vi "Async Loop.vi"(1 "RT Data":T1={"Device ref"=0, "Scan Period (uSec)"=10000, "Device Channels"={"Status"={"BD Refs"=[], "Length"=0, "FIFO Index"=0, "Data"=[]}, "Command"={"BD Refs"=[], "Data"=[], "Length"=0, "FIFO Index"=0}}, "Local Chassis"=[], "EtherCAT Masters"=[], "Async"={"Status"=refnum, "Command"=refnum, "Input FIFO"=refnum, "Input FIFO buffer"=[], "Output FIFO"=refnum, "Output FIFO buffer"=[], "Async VI Ref"=refnum}, "ECAT Reconfig"={"Reconfig Module Found"=FALSE, "VI Ref"=refnum, "Status"=refnum}, "Device Error"={"status"=FALSE, "code"=0, "source"=""}, "DeviceName"="", "PCLSync?"=FALSE} {"Device Channels"."Status"."BD Refs"."Data Reference" format="%.0x"; "Device Channels"."Command"."BD Refs"."Data Reference" format="%.0x"; "Local Chassis"."FPGA"."VS ref" format="%.0x"; "Local Chassis"."RSI Modules"."VS ref" format="%.0x"; "Local Chassis"."VS ref" format="%.0x"; "Device ref" format="%.0x"; "EtherCAT Masters"."REM IO ECAT Slaves"."VS ref" format="%.0x"; "EtherCAT Masters"."Generic EtherCAT Slaves"."VS ref" format="%.0x"; "EtherCAT Masters"."VS ref" format="%.0x"; "EtherCAT Masters"."EtherCAT Slaves"."FPGA"."VS ref" format="%.0x"; "EtherCAT Masters"."EtherCAT Slaves"."RSI Modules"."VS ref" format="%.0x"; "EtherCAT Masters"."EtherCAT Slaves"."VS ref" format="%.0x"}) -> ()   [LabVIEW 2020, in "SEECD Engine.lvlib"]
uses:
  SEECD Engine.lvlib
  <vilib>/Platform/TimedLoop/XDataNode/XDataNode.xnode
  <vilib>/Platform/TimedLoop/XDataNode/nitl_modes.ctl
  <vilib>/Platform/TimedLoop/XDataNode/XDNodeRunTimeDep.lvlib
  <vilib>/Platform/TimedLoop/XDataNode/wakeup.ctl
  <vilib>/Platform/TimedLoop/XDataNode/timing_clust.ctl
  <vilib>/NI VeriStand/Custom Device API/Custom Device API.lvlib
  <vilib>/NI VeriStand/Custom Device API/Custom Device Timed Loop Priority.ctl
  Type Defs/Async State.ctl
  Shared/Globals/String Constants.vi
  Shared/SEECD Shared.lvlib
  Type Defs/RW Case.ctl
  Type Defs/Async Command.ctl
  <vilib>/Platform/TimedLoop/XDataNode/loadnilvce.vi
  <vilib>/NI VeriStand/Custom Device Tools/Custom Device Utility Library/Custom Device Utility Library.lvlib
  <vilib>/NI VeriStand/Custom Device API/Custom Device Item Ref.ctl
  Includes/Modules.lvlibp/RSI Module/RSI Module.lvclass
  <vilib>/NI VeriStand/Custom Device API/Data Reference.ctl
  <vilib>/NI VeriStand/Custom Device API/Block Data Reference.ctl
  Type Defs/Input Data.ctl
  Type Defs/Output Data.ctl
  Includes/Modules.lvlibp/RSI Module/Channel Type.ctl
  Type Defs/RSI Module Data.ctl
  Type Defs/FPGA Data.ctl
  Type Defs/Local Chassis Data.ctl
  Type Defs/EtherCAT Slave Data.ctl
  Type Defs/EtherCAT Master Data.ctl
  Type Defs/RT Data.ctl
  Type Defs/Async Status.ctl
  Shared/Type Defs/UDV Data Type.ctl
  Shared/Type Defs/FXP Config.ctl
  Type Defs/UDV Data.ctl
  Includes/Modules.lvlibp/RSI Module/Module Models.ctl
  Type Defs/Module Config Data.ctl
  Type Defs/Async Data.ctl
  Type Defs/ECAT Reconfig State.ctl
  Type Defs/ECAT Reconfig Status.ctl
  Type Defs/ECAT Reconfig Data.ctl
  Type Defs/Device Channels.ctl
  Type Defs/Mixed IO.ctl
  Type Defs/Open Module IOVs.ctl
  Type Defs/Mod Size Indexes.ctl
  Type Defs/Generic ECAT Slave IOV Cluster.ctl
  Type Defs/Generic ECAT Slave Data Cluster.ctl
  Type Defs/Generic ECAT Slave RT-Data-Array.ctl
  Type Defs/REM IO ECAT Slave IOV Cluster.ctl
  Type Defs/REM IO ECAT Slave Data Cluster.ctl
  Type Defs/REM IO ECAT Slave RT-Data-Array.ctl
types:
  T1 = typedef "SEECD Engine.lvlib/RT Data.ctl" = cluster{"Device ref":T2, "Scan Period (uSec)":u32, "Device Channels":T3, "Local Chassis":T8[], "EtherCAT Masters":T20[], "Async":T28, "ECAT Reconfig":T29, "Device Error":errorcluster, "DeviceName":string, "PCLSync?":bool}
  T2 = typedef "Custom Device API.lvlib/Custom Device Item Ref.ctl" = u64
  T3 = typedef "SEECD Engine.lvlib/Device Channels.ctl" = cluster{"Status":T4, "Command":T7}
  T4 = typedef "SEECD Engine.lvlib/Output Data.ctl" = cluster{"BD Refs":T5[], "Length":i32, "FIFO Index":i32, "Data":dbl[]}
  T5 = typedef "Custom Device API.lvlib/Block Data Reference.ctl" = cluster{"Data Reference":T6, "Offset":u64, "Length":u64}
  T6 = typedef "Custom Device API.lvlib/Data Reference.ctl" = i32
  T7 = typedef "SEECD Engine.lvlib/Input Data.ctl" = cluster{"BD Refs":T5[], "Data":dbl[], "Length":i32, "FIFO Index":i32}
  T8 = typedef "SEECD Engine.lvlib/Local Chassis Data.ctl" = cluster{"VS ref":T2, "RSI Modules":T9[], "FPGA":T15[], "Input Mod Size Idxs":T19, "Output Modules":i32[], "MixedIO Mod Size Idxs":T19}
  T9 = typedef "SEECD Engine.lvlib/RSI Module Data.ctl" = cluster{"VS ref":T2, "IOV ref":refnum<k21>, "Open Mod refs":T10, "Module DVR":refnum<data-value>, "Slot":u32, "Model":T11, "Channel Type":T12, "EtherCAT?":bool, "CDInput Data":T7, "CDOutput Data":T4, "Module Config Data":T13, "Mixed IO":T14}
  T10 = typedef "SEECD Engine.lvlib/Open Module IOVs.ctl" = cluster{"Analog Read":refnum<k21>, "Digital Read":refnum<k21>, "Analog Write":refnum<k21>, "Digital Write":refnum<k21>}
  T11 = typedef "Modules.lvlibp/RSI Module.lvclass/Module Models.ctl" = enum16{"Empty", "NI 9201", "NI 9203", "NI 9205", "NI 9206", "NI 9207", "NI 9208", "NI 9209", "NI 9210", "NI 9211", "NI 9212", "NI 9213", "NI 9214", "NI 9215", "NI 9216", "NI 9217", "NI 9219", "NI 9220", "NI 9221", "NI 9222", "NI 9223", "NI 9224", "NI 9225", "NI 9226", "NI 9227", "NI 9228", "NI 9229", "NI 9233", "NI 9234", "NI 9235", "NI 9236", "NI 9237", "NI 9239", "NI 9242", "NI 9244", "NI 9253", "NI 9263", "NI 9264", "NI 9265", "NI 9266", "NI 9269", "NI 9344", "NI 9350", "NI 9375", "NI 9401", "NI 9402", "NI 9403", "NI 9411", "NI 9421", "NI 9422", "NI 9423", "NI 9425", "NI 9426", "NI 9435", "NI 9436", "NI 9437", "NI 9472", "NI 9474", "NI 9475", "NI 9476", "NI 9477", "NI 9478", "NI 9481", "NI 9482", "NI 9485"}
  T12 = typedef "Modules.lvlibp/RSI Module.lvclass/Channel Type.ctl" = enum16{"Analog", "Digital"}
  T13 = typedef "SEECD Engine.lvlib/Module Config Data.ctl" = cluster{"Configurable?":bool, "Config Block Data Refs":T5[], "Config Data DVR":refnum<data-value>, "Previous Values":dbl[], "Local Reconfig VI Ref":refnum<vi>}
  T14 = typedef "SEECD Engine.lvlib/Mixed IO.ctl" = cluster{"Input Channel Indices":i32[], "Input Buffer":dbl[]}
  T15 = typedef "SEECD Engine.lvlib/FPGA Data.ctl" = cluster{"VS ref":T2, "IOV ref":refnum<k21>, "FPGA Target":enum16{"Local", "EtherCAT"}, "Product Code":u32, "Bitfile Signature":string, "Bitfile Path (RT)":path, "FPGA Session":u32, "Input Data":T7, "Output Data":T4, "UDVs":cluster{"From FPGA":T16[], "To FPGA":T16[]}}
  T16 = typedef "SEECD Engine.lvlib/UDV Data.ctl" = cluster{"VS ref":T2, "IOV Ref":refnum<k21>, "Name":string, "UDV Data Type":T17, "Supported Type?":bool, "FXP Config":T18, "FXP VI Ref":refnum<vi>}
  T17 = typedef "SEECD Shared.lvlib/UDV Data Type.ctl" = enum16{"Boolean", "Fixed Point", "Int8", "Int16", "Int32", "Int64", "U32 Bit Field", "UInt8", "UInt16", "UInt32", "UInt64", "Other", "DBL", "SGL"}
  T18 = typedef "SEECD Shared.lvlib/FXP Config.ctl" = cluster{"signed":bool, "size":u32, "integersize":i32}
  T19 = typedef "SEECD Engine.lvlib/Mod Size Indexes.ctl" = cluster{"4":i32[], "8":i32[], "16":i32[], "32":i32[], "other":i32[]}
  T20 = typedef "SEECD Engine.lvlib/EtherCAT Master Data.ctl" = cluster{"VS ref":T2, "IOV ref":refnum<k21>, "Master ID":u32, "Cyclic Data Bandwidth":u32, "EtherCAT Slaves":T21[], "Generic EtherCAT Slaves":T22, "REM IO ECAT Slaves":T25}
  T21 = typedef "SEECD Engine.lvlib/EtherCAT Slave Data.ctl" = cluster{"VS ref":T2, "IOV ref":refnum<k21>, "Position Address":u16, "RSI Modules":T9[], "FPGA":T15[], "Input Mod Size Idxs":T19, "Output Modules":i32[], "MixedIO Mod Size Idxs":T19}
  T22 = typedef "SEECD Engine.lvlib/Generic ECAT Slave RT-Data-Array.ctl" = T23[]
  T23 = typedef "SEECD Engine.lvlib/Generic ECAT Slave Data Cluster.ctl" = cluster{"VS ref":T2, "IOV ref":refnum<k21>, "Position Address":u16, "I/O Imput Vars ":T24[], "I/O Output Vars":T24[], "I/O Input Data":T7, "I/O Output Data":T4, "Distributed Clock":bool}
  T24 = typedef "SEECD Engine.lvlib/Generic ECAT Slave IOV Cluster.ctl" = cluster{"VS ref":T2, "IOV Ref":refnum<k21>, "Name":string, "UDV Data Type":T17}
  T25 = typedef "SEECD Engine.lvlib/REM IO ECAT Slave RT-Data-Array.ctl" = T26[]
  T26 = typedef "SEECD Engine.lvlib/REM IO ECAT Slave Data Cluster.ctl" = cluster{"VS ref":T2, "IOV ref":refnum<k21>, "Position Address":u16, "I/O Imput Vars ":T27[], "I/O Output Vars":T27[], "I/O Input Data":T7, "I/O Output Data":T4}
  T27 = typedef "SEECD Engine.lvlib/REM IO ECAT Slave IOV Cluster.ctl" = cluster{"VS ref":T2, "IOV Ref":refnum<k21>, "Name":string, "UDV Data Type":T17, "Scaling Factor":dbl}
  T28 = typedef "SEECD Engine.lvlib/Async Data.ctl" = cluster{"Status":refnum<queue>, "Command":refnum<queue>, "Input FIFO":refnum<k33>, "Input FIFO buffer":dbl[], "Output FIFO":refnum<k33>, "Output FIFO buffer":dbl[], "Async VI Ref":refnum<vi>}
  T29 = typedef "SEECD Engine.lvlib/ECAT Reconfig Data.ctl" = cluster{"Reconfig Module Found":bool, "VI Ref":refnum<vi>, "Status":refnum<queue>}
  T30 = typedef "SEECD Engine.lvlib/Async State.ctl" = enum16{"Not running", "Waiting on start cmd", "Running", "Paused", "Stopped"}
  T31 = typedef "SEECD Engine.lvlib/Async Command.ctl" = enum16{"None", "Start", "Stop"}
  T32 = typedef "Custom Device API.lvlib/Custom Device Timed Loop Priority.ctl" = enum32{"Low", "Medium", "High"}
  T33 = typedef "SEECD Engine.lvlib/RW Case.ctl" = enum16{"Inline read", "Inline write", "Async - Inline loop read", "Async - Inline loop write", "Async loop (read/write)"}
  T34 = typedef "XDNodeRunTimeDep.lvlib/timing_clust.ctl" = cluster{"Expected End [f-1]":u64, "Actual End [f-1]":u64, "Finished Late? [f-1]":bool, "Expected End [i-1]":u64, "Actual End [i-1]":u64, "Finished Late? [i-1]":bool, "Expected Start [i]":u64, "Actual Start [i]":u64, "Expected Start [f]":u64, "Actual Start [f]":u64, "Source Name":string, "Structure Name":string, "Period":i64, "Deadline":i64, "Offset":i64, "Start":i64, "Priority":i32, "Timeout":i32, "Mode":T35, "Wakeup Reason":T36, "Error":errorcluster, "Source Type":string, "Secondary Source Type":string, "Global End Time":u64, "Global Start Time":u64, "Frame Duration":u64, "Iteration Duration":u64, "Assigned CPU":i32, "I/O Scan Engine Mode":u32}
  T35 = typedef "XDNodeRunTimeDep.lvlib/nitl_modes.ctl" = enum32{"No Change", "Process missed periods, maintain original phase", "Discard missed periods, maintain original phase", "Process missed periods, ignore original phase", "Discard missed periods, ignore original phase"}
  T36 = typedef "XDNodeRunTimeDep.lvlib/wakeup.ctl" = enum32{"Normal", "Aborted", "Asynchronous wakeup", "Timing source error", "Timed loop error", "Timeout"}
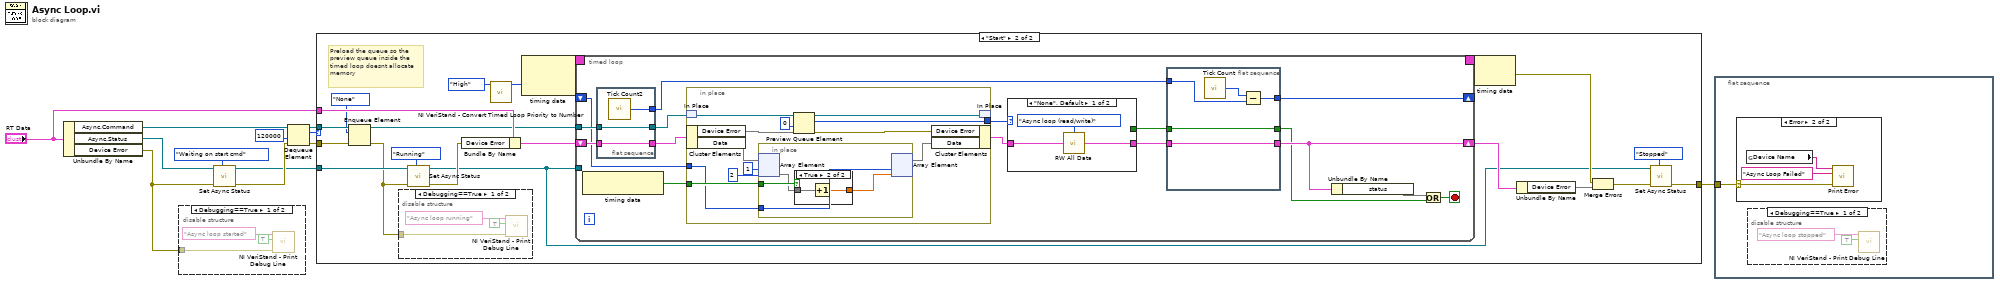
[diagram p0: block diagram]
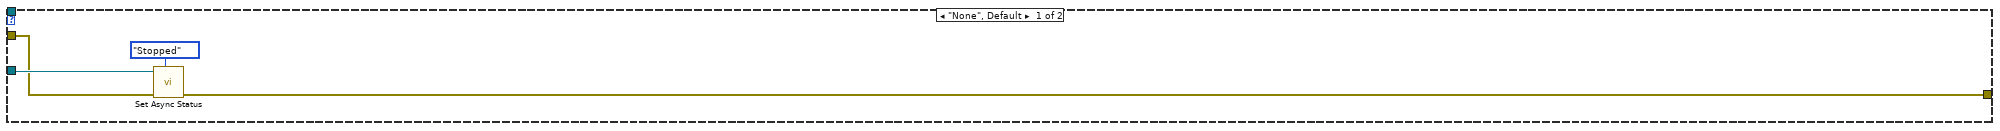
[diagram p5: hidden frame]
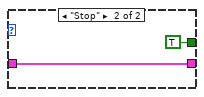
[diagram p7: hidden frame]
diagram:
  n1 = Unbundle By Name("RT Data") -> ("Async.Command"=w7:refnum<queue>, "Async.Status"=w9:refnum<queue>, "Device Error"=w1:errorcluster)
  n2 = disable-structure shown="Debugging==True" {
    disable-tunnel: w1 -> [w14 _]
    frame condition #0 {
      n3 = call <vilib>:"NI VeriStand - Print Debug Line.vi"("error in (no error)"=w14, "Add to log file? (F)"=TRUE, "Message"="Async loop started" ("String to write")) -> ()  [unwired: 8 in, 1 out]
    }
    frame condition #1 (active) {
    }
  }
  n4 = call "Set Async Status.vi"("State"=Async_State."Waiting on start cmd", "error in (no error)"=w1, "Status in"=w9) -> ("error out"=w6:errorcluster, "Status out"=w4:refnum<queue>)  [unwired: 7 in]
  n5 = Dequeue Element(queue=w7, timeout in ms (-1)=120000, error in (no error)=w6) -> (queue out=w5:refnum<queue>, element=w10:T31, error out=w3:errorcluster)  [unwired: 1 out]
  n6 = case shown="\"Start\"" w10 {
    tunnel: "RT Data" -> [_ w34]
    tunnel: w5 -> [_ w23]
    tunnel: w4 -> [w18 w36]
    tunnel: w3 -> [w17 w35]
    tunnel: [w16 w30] -> w2
    frame "None", Default {
      n7 = call "Set Async Status.vi"("State"=Async_State."Stopped", "error in (no error)"=w17, "Status in"=w18) -> ("error out"=w16:errorcluster)  [unwired: 7 in, 1 out]
    }
    frame "Start" {
      # "Preload the queue so the preview queue inside the timed loop doesnt allocate memory"
      n8 = Enqueue Element(queue=w23, element=Async_Command."None", error in (no error)=w35) -> (queue out=w22:refnum<queue>, error out=w20:errorcluster)  [unwired: 1 in, 1 out]
      n9 = disable-structure shown="Debugging==True" {
        disable-tunnel: w20 -> [w42 _]
        frame condition #0 {
          n10 = call <vilib>:"NI VeriStand - Print Debug Line.vi"("error in (no error)"=w42, "Add to log file? (F)"=TRUE, "Message"="Async loop running" ("String to write")) -> ()  [unwired: 8 in, 1 out]
        }
        frame condition #1 (active) {
        }
      }
      n11 = call "Set Async Status.vi"("State"=Async_State."Running", "error in (no error)"=w20, "Status in"=w36) -> ("error out"=w26:errorcluster, "Status out"=w24:refnum<queue>)  [unwired: 7 in]
      n12 = Bundle By Name(cluster=w34, "Device Error"=w26) -> (w33:T1)
      n13 = call <vilib>:"NI VeriStand - Convert Timed Loop Priority to Number.vi"("Priority"=Custom_Device_Timed_Loop_Priority."High") -> ("Numeric Priority"=w37:i32)  [unwired: 10 in]
      n14 = node-c288(w37) -> (w40:T34)  [unwired: 1 in]
      n15 = timed-loop {
        timing: w40 -> [_]
        timing-out: [_] -> w39
        shift-right: [w54] -> w31
        shift-left: w33 -> [w48]
        tunnel: w22 -> [w50]
        tunnel: w24 -> [_]
        shift-right: [w57] -> _
        shift-left: _ -> [w45]
        stop <- w58 stop-if-true
        n16 = node-c288() -> (w46:bool)  [unwired: 1 in]
        n17 = flat-sequence {
          tunnel: w50 -> [w62]
          tunnel: [w62] -> w44
          tunnel: [w61] -> w49
          tunnel: w48 -> [w61]
          tunnel: [w60] -> w47
          frame #0 {
            n18 = call "Tick Count2"() -> ("Tick Count(uSec)"=w60:u32)
          }
        }
        n19 = in-place {
          in-place-border: [w81] -> w55
          in-place-border: w46 -> [w77]
          in-place-border: w45 -> [w76]
          n20 = in-place-match #1(w44) -> (w74:refnum<queue>)
          n21 = in-place-cluster #2(w49) -> ("Device Error"=w83, "Data"=w80)
          n22 = in-place {
            in-place-border: w77 -> [w88]
            in-place-border: w76 -> [w85]
            n23 = in-place-array #3(w80, 1, 2) -> (w87)  [unwired: 1 out]
            n24 = case shown="True" w88 {
              tunnel: w87 -> [w89 w91]
              tunnel: [w89 w90] -> w86
              frame False {
              }
              frame True {
                n25 = Increment(x=w91) -> (x+1=w90:dbl)
              }
            }
            n26 = in-place-array #3(w85, w86) -> (w75)  [unwired: 2 out]
          }
          n27 = Preview Queue Element(queue=w74, timeout in ms (-1)=0, error in (no error)=w83) -> (queue out=w73:refnum<queue>, element=w81:T31, error out=w82:errorcluster)  [unwired: 1 out]
          n28 = in-place-cluster #2("Device Error"=w82, "Data"=w75) -> (w56:cluster{})
          n29 = in-place-match #1(w73) -> ()  [unwired: 1 out]
        }
        n30 = case shown="\"None\", Default" w55 {
          tunnel: [_ TRUE] -> w51
          tunnel: w56 -> [w70 w71]
          tunnel: [w68 w71] -> w53
          frame "None", Default {
            n31 = call "RW All Data.vi"("R/W Case"=RW_Case."Async loop (read/write)", "RT Data in"=w70) -> ("RT Data out"=w68:T1)  [unwired: 13 in]
          }
          frame "Stop" {
          }
        }
        n32 = flat-sequence {
          tunnel: [w67] -> w57
          tunnel: w47 -> [w66]
          tunnel: [w64] -> w54
          tunnel: w53 -> [w64]
          tunnel: [w63] -> w52
          tunnel: w51 -> [w63]
          frame #0 {
            n33 = call "Tick Count"() -> ("Tick Count(uSec)"=w65:u32)
            n34 = Subtract(x=w65, y=w66) -> (x-y=w67:u32)
          }
        }
        n35 = Unbundle By Name(w54) -> ("status"=w59)
        n36 = Or(x=w59, y=w52) -> (x .or. y?=w58:bool)
      }
      n37 = node-c288(w39) -> (w29:errorcluster)
      n38 = Unbundle By Name(w31) -> ("Device Error"=w28)
      n39 = Merge Errors(w29, w28) -> (w27:errorcluster)
      n40 = call "Set Async Status.vi"("State"=Async_State."Stopped", "error in (no error)"=w27, "Status in"=w24) -> ("error out"=w30:errorcluster)  [unwired: 7 in, 1 out]
    }
  }
  n41 = flat-sequence {
    tunnel: w2 -> [w100]
    frame #0 {
      n42 = case shown="Error" w100 {
        selector: w100 -> [_ w103]
        frame No Error {
        }
        frame Error {
          n43 = global read "String Constants.vi" "Device Name"() -> (w105:string)
          n44 = call "Print Error.vi"("error in (no error)"=w103, "Note (empty)"="Async Loop Failed", "Your code's public name"=w105) -> ()  [unwired: 7 in, 1 out]
        }
      }
      n45 = disable-structure shown="Debugging==True" {
        frame condition #0 {
          n46 = call <vilib>:"NI VeriStand - Print Debug Line.vi"("Add to log file? (F)"=TRUE, "Message"="Async loop stopped" ("String to write")) -> ()  [unwired: 9 in, 1 out]
        }
        frame condition #1 (active) {
        }
      }
    }
  }
